vi "labview project.vi"() -> ()   [LabVIEW 2018]
panel:
  out "Fire suppression system":bool
  out "A/C":bool
  out "FAN":bool
  out "Thermometer 2":dbl(slide) scale=0.0..100.0
  in  "Thermometer":dbl(slide) scale=0.0..100.0
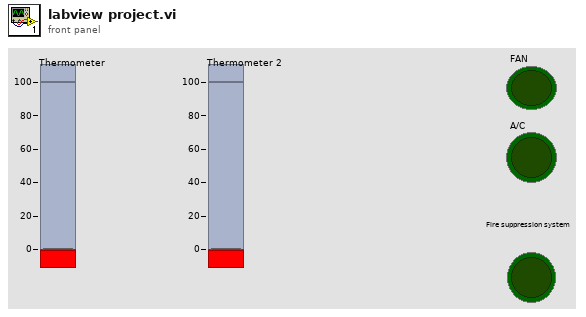
[diagram p1: front panel]
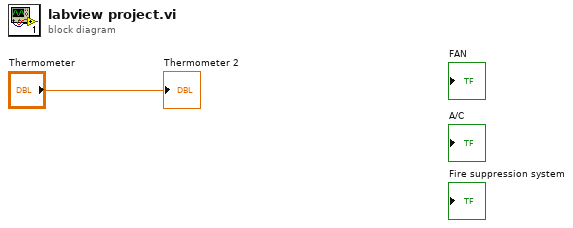
[diagram p0: block diagram]
diagram:
  "Thermometer 2" <- "Thermometer"
